vi "Process Messages.vi"(8 "error in (no error)":errorcluster, 11 "Mixer in":refnum<class "Mixer.lvclass">) -> (0 "error out":errorcluster, 3 "Mixer out":refnum<class "Mixer.lvclass">)   [LabVIEW 2019, in "Mixer.lvclass"]
uses:
  Mixer.lvclass
  Mixer.lvclass/Mixer.ctl
  Packed Libraries/Messaging.lvlibp
  Packed Libraries/Audio Processing.lvlibp
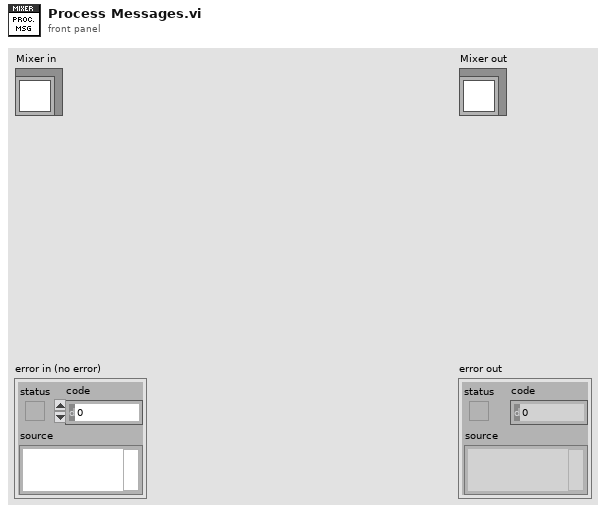
[diagram p1: front panel]
types:
  T1 = typedef "Messaging.lvlibp/Message Cluster.ctl" = cluster{"Event":string, "Source":string, "Target":string, "Data":variant}
  T2 = typedef "Audio Processing.lvlibp/Value Properties.ctl" = cluster{"Lower":dbl, "Upper":dbl, "Default":dbl, "Increment":dbl}
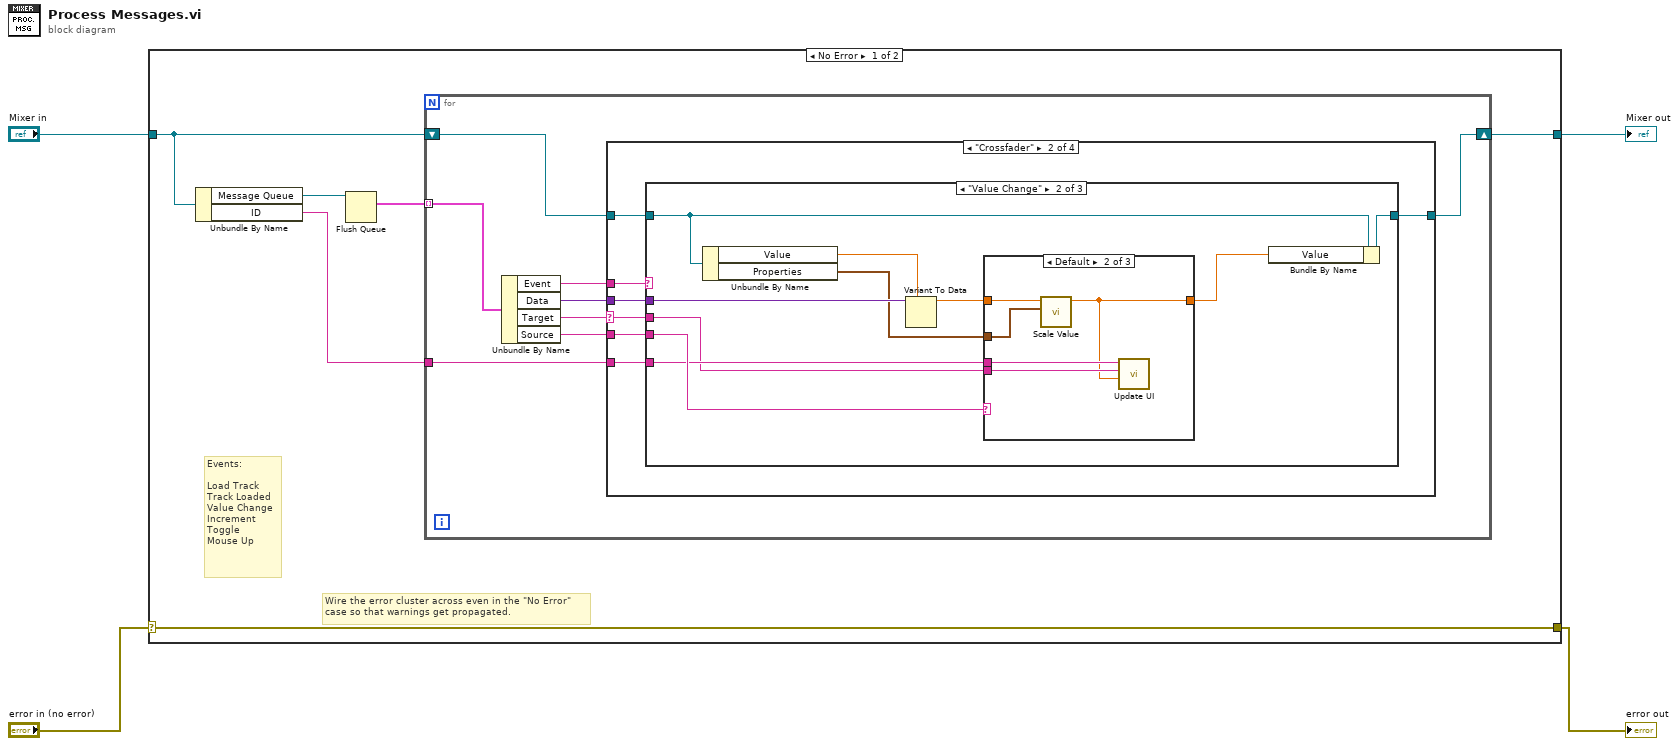
[diagram p0: block diagram]
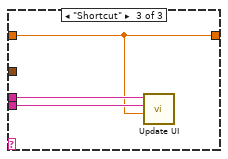
[diagram p5: hidden frame]
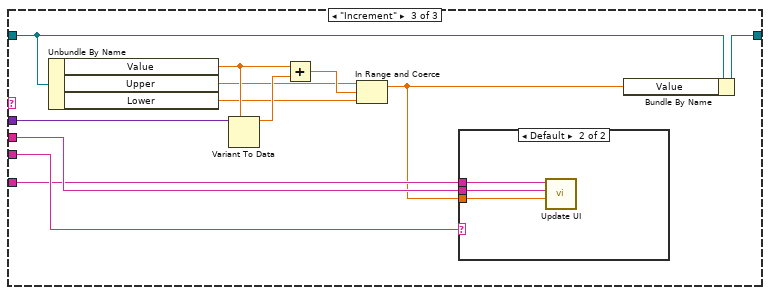
[diagram p6: hidden frame]
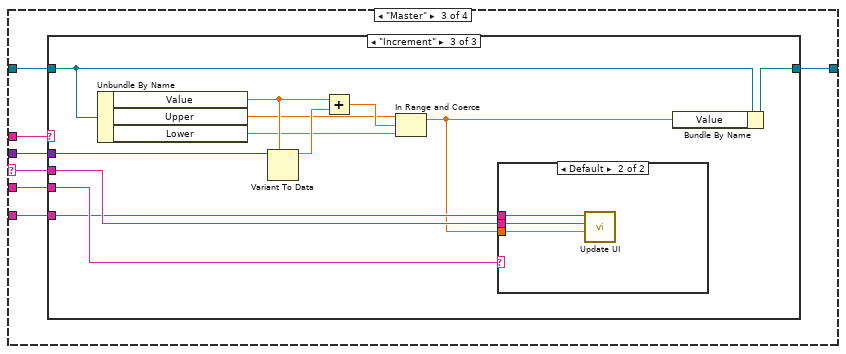
[diagram p8: hidden frame]
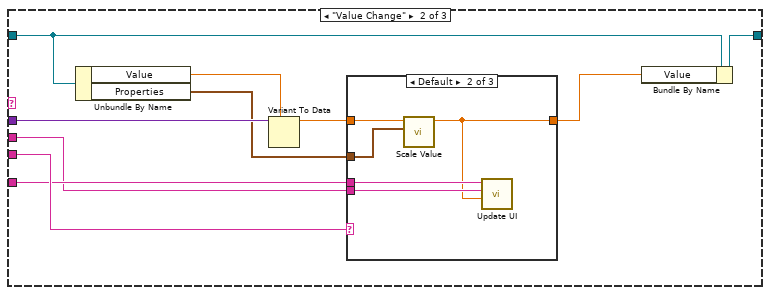
[diagram p10: hidden frame]
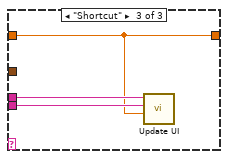
[diagram p12: hidden frame]
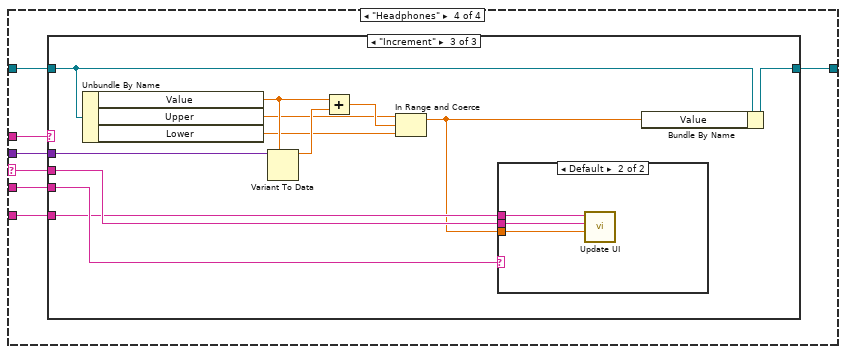
[diagram p14: hidden frame]
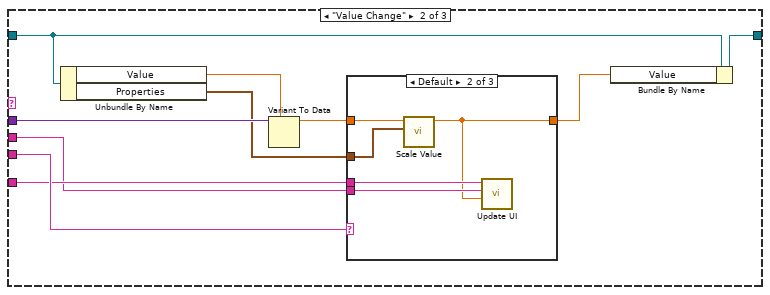
[diagram p16: hidden frame]
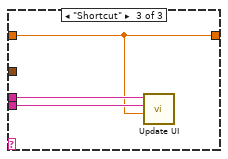
[diagram p18: hidden frame]
diagram:
  n1 = case shown="No Error" "error in (no error)" {
    selector: "error in (no error)" -> [w10 w147]
    tunnel: [w10 w147] -> w2
    tunnel: [w5 w146] -> w1
    tunnel: "Mixer in" -> [w9 w146]
    frame No Error {
      # "Events:\n\nLoad Track\nTrack Loaded\nValue Change\nIncrement\nToggle\nMouse Up"
      # "Wire the error cluster across even in the \"No Error\"\ncase so that warnings get propagated."
      n2 = Unbundle By Name(w9) -> ("Message Queue"=w8:refnum<queue>, "ID"=w6:string)
      n3 = Flush Queue(queue=w8) -> (remaining elements=w7:T1[])  [unwired: 1 in, 2 out]
      n4 = for {
        shift-right: [w17] -> w5
        shift-left: w9 -> [w18]
        tunnel: w7 -> [w16] mode=indexing
        tunnel: w6 -> [w11]
        n5 = Unbundle By Name(w16) -> ("Event"=w13:string, "Data"=w14:variant, "Target"=w15:string, "Source"=w12:string)
        n6 = case shown="\"Crossfader\"" w15 {
          selector: w15 -> [_ w21 w65 w107]
          tunnel: w18 -> [w19 w24 w68 w110]
          tunnel: [w19 w25 w62 w104] -> w17
          tunnel: w14 -> [_ w23 w66 w108]
          tunnel: w13 -> [_ w26 w67 w109]
          tunnel: w12 -> [_ w22 w64 w106]
          tunnel: w11 -> [_ w20 w63 w105]
          frame Default {
          }
          frame "Crossfader" {
            n7 = case shown="\"Value Change\"" w26 {
              tunnel: [w27 w34 w56] -> w25
              tunnel: w24 -> [w27 w35 w57]
              tunnel: w23 -> [_ w36 w58]
              tunnel: w22 -> [_ w32 w55]
              tunnel: w21 -> [_ w30 w54]
              tunnel: w20 -> [_ w31 w53]
              frame Default {
              }
              frame "Value Change" {
                n8 = Unbundle By Name(w35) -> ("Value"=w37:dbl, "Properties"=w28:T2)
                n9 = Variant To Data(type=w37, Variant=w36) -> (data=w33:dbl)  [unwired: 1 in, 1 out]
                n10 = case shown="Default" w32 {
                  tunnel: w33 -> [w38 w41 w44]
                  tunnel: w30 -> [_ w43 w46]
                  tunnel: w31 -> [_ w42 w45]
                  tunnel: [w38 w39 w44] -> w29
                  tunnel: w28 -> [_ w40 _]
                  frame "UI" {
                  }
                  frame Default {
                    n11 = call "Scale Value.vi"("Properties"=w40, "Value"=w41) -> ("Scaled Value"=w39:dbl)  [unwired: 9 in]
                    n12 = call "Update UI.vi"("Data"=w39, "Target"=w43, "ID"=w42) -> ()  [unwired: 8 in, 1 out]
                  }
                  frame "Shortcut" {
                    n13 = call "Update UI.vi"("Data"=w44, "Target"=w46, "ID"=w45) -> ()  [unwired: 8 in, 1 out]
                  }
                }
                n14 = Bundle By Name(cluster=w35, "Value"=w29) -> (w34:refnum<class "Mixer.lvclass">)
              }
              frame "Increment" {
                n15 = Unbundle By Name(w57) -> ("Value"=w52:dbl, "Upper"=w49:dbl, "Lower"=w48:dbl)
                n16 = Variant To Data(type=w52, Variant=w58) -> (data=w51:dbl)  [unwired: 1 in, 1 out]
                n17 = Add(x=w52, y=w51) -> (x+y=w50:dbl)
                n18 = In Range and Coerce(upper limit=w49, x=w50, lower limit=w48) -> (coerced(x)=w47:dbl)  [unwired: 1 out]
                n19 = case shown="Default" w55 {
                  tunnel: w47 -> [_ w61]
                  tunnel: w54 -> [_ w60]
                  tunnel: w53 -> [_ w59]
                  frame "UI" {
                  }
                  frame Default {
                    n20 = call "Update UI.vi"("Data"=w61, "Target"=w60, "ID"=w59) -> ()  [unwired: 8 in, 1 out]
                  }
                }
                n21 = Bundle By Name(cluster=w57, "Value"=w47) -> (w56:refnum<class "Mixer.lvclass">)
              }
            }
          }
          frame "Master" {
            n22 = case shown="\"Increment\"" w67 {
              tunnel: [w69 w76 w98] -> w62
              tunnel: w68 -> [w69 w77 w99]
              tunnel: w66 -> [_ w78 w100]
              tunnel: w64 -> [_ w74 w97]
              tunnel: w65 -> [_ w72 w96]
              tunnel: w63 -> [_ w73 w95]
              frame Default {
              }
              frame "Value Change" {
                n23 = Unbundle By Name(w77) -> ("Value"=w79:dbl, "Properties"=w70:T2)
                n24 = Variant To Data(type=w79, Variant=w78) -> (data=w75:dbl)  [unwired: 1 in, 1 out]
                n25 = case shown="Default" w74 {
                  tunnel: w75 -> [w80 w83 w86]
                  tunnel: w72 -> [_ w85 w88]
                  tunnel: w73 -> [_ w84 w87]
                  tunnel: [w80 w81 w86] -> w71
                  tunnel: w70 -> [_ w82 _]
                  frame "UI" {
                  }
                  frame Default {
                    n26 = call "Scale Value.vi"("Properties"=w82, "Value"=w83) -> ("Scaled Value"=w81:dbl)  [unwired: 9 in]
                    n27 = call "Update UI.vi"("Data"=w81, "Target"=w85, "ID"=w84) -> ()  [unwired: 8 in, 1 out]
                  }
                  frame "Shortcut" {
                    n28 = call "Update UI.vi"("Data"=w86, "Target"=w88, "ID"=w87) -> ()  [unwired: 8 in, 1 out]
                  }
                }
                n29 = Bundle By Name(cluster=w77, "Value"=w71) -> (w76:refnum<class "Mixer.lvclass">)
              }
              frame "Increment" {
                n30 = Unbundle By Name(w99) -> ("Value"=w94:dbl, "Upper"=w91:dbl, "Lower"=w90:dbl)
                n31 = Variant To Data(type=w94, Variant=w100) -> (data=w93:dbl)  [unwired: 1 in, 1 out]
                n32 = Add(x=w94, y=w93) -> (x+y=w92:dbl)
                n33 = In Range and Coerce(upper limit=w91, x=w92, lower limit=w90) -> (coerced(x)=w89:dbl)  [unwired: 1 out]
                n34 = case shown="Default" w97 {
                  tunnel: w89 -> [_ w103]
                  tunnel: w96 -> [_ w102]
                  tunnel: w95 -> [_ w101]
                  frame "UI" {
                  }
                  frame Default {
                    n35 = call "Update UI.vi"("Data"=w103, "Target"=w102, "ID"=w101) -> ()  [unwired: 8 in, 1 out]
                  }
                }
                n36 = Bundle By Name(cluster=w99, "Value"=w89) -> (w98:refnum<class "Mixer.lvclass">)
              }
            }
          }
          frame "Headphones" {
            n37 = case shown="\"Increment\"" w109 {
              tunnel: [w111 w118 w140] -> w104
              tunnel: w110 -> [w111 w119 w141]
              tunnel: w108 -> [_ w120 w142]
              tunnel: w106 -> [_ w116 w139]
              tunnel: w107 -> [_ w114 w138]
              tunnel: w105 -> [_ w115 w137]
              frame Default {
              }
              frame "Value Change" {
                n38 = Unbundle By Name(w119) -> ("Value"=w121:dbl, "Properties"=w112:T2)
                n39 = Variant To Data(type=w121, Variant=w120) -> (data=w117:dbl)  [unwired: 1 in, 1 out]
                n40 = case shown="Default" w116 {
                  tunnel: w117 -> [w122 w125 w128]
                  tunnel: w114 -> [_ w127 w130]
                  tunnel: w115 -> [_ w126 w129]
                  tunnel: [w122 w123 w128] -> w113
                  tunnel: w112 -> [_ w124 _]
                  frame "UI" {
                  }
                  frame Default {
                    n41 = call "Scale Value.vi"("Properties"=w124, "Value"=w125) -> ("Scaled Value"=w123:dbl)  [unwired: 9 in]
                    n42 = call "Update UI.vi"("Data"=w123, "Target"=w127, "ID"=w126) -> ()  [unwired: 8 in, 1 out]
                  }
                  frame "Shortcut" {
                    n43 = call "Update UI.vi"("Data"=w128, "Target"=w130, "ID"=w129) -> ()  [unwired: 8 in, 1 out]
                  }
                }
                n44 = Bundle By Name(cluster=w119, "Value"=w113) -> (w118:refnum<class "Mixer.lvclass">)
              }
              frame "Increment" {
                n45 = Unbundle By Name(w141) -> ("Value"=w136:dbl, "Upper"=w133:dbl, "Lower"=w132:dbl)
                n46 = Variant To Data(type=w136, Variant=w142) -> (data=w135:dbl)  [unwired: 1 in, 1 out]
                n47 = Add(x=w136, y=w135) -> (x+y=w134:dbl)
                n48 = In Range and Coerce(upper limit=w133, x=w134, lower limit=w132) -> (coerced(x)=w131:dbl)  [unwired: 1 out]
                n49 = case shown="Default" w139 {
                  tunnel: w131 -> [_ w145]
                  tunnel: w138 -> [_ w144]
                  tunnel: w137 -> [_ w143]
                  frame "UI" {
                  }
                  frame Default {
                    n50 = call "Update UI.vi"("Data"=w145, "Target"=w144, "ID"=w143) -> ()  [unwired: 8 in, 1 out]
                  }
                }
                n51 = Bundle By Name(cluster=w141, "Value"=w131) -> (w140:refnum<class "Mixer.lvclass">)
              }
            }
          }
        }
      }
    }
    frame Error {
    }
  }
  "error out" <- w2
  "Mixer out" <- w1
